vi "From CSV File.vi"(8 "error in (no error)":errorcluster, 9 "Path":path, 10 "engine in":refnum<class "engine configuration.lvclass">, 11 "module editor node in":refnum<class "module editor node.lvclass">) -> (0 "error out":errorcluster, 1 "Update":bool, 2 "engine out":refnum<class "engine configuration.lvclass">, 3 "module editor node out":refnum<class "module editor node.lvclass">)   [LabVIEW 2014, in "PL Framework Configuration Tool.lvlib" / "module editor node.lvclass"]
uses:
  module editor node.lvclass
  <vilib>/NI/Module Execution Interface/Engine Configuration/engine configuration.lvclass
  <vilib>/NI/Tag Bus Module Framework/module configuration/TBM module configuration.lvclass
  <vilib>/NI/Configuration Framework/serializable configuration/NISE_CEF_serializable configuration.lvclass
panel:
  in  "type (empty)":string[][](array[string])
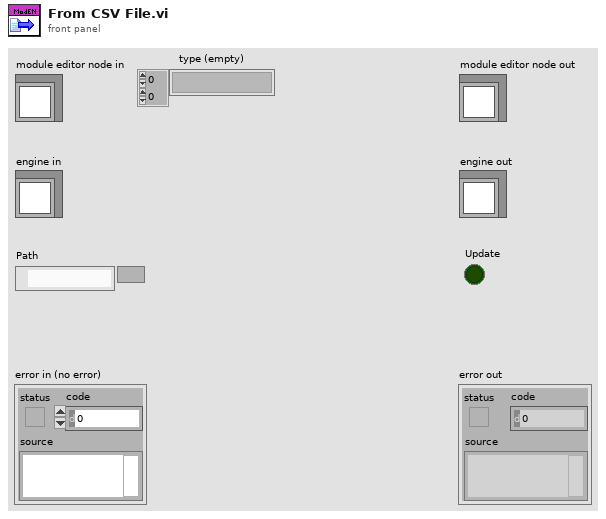
[diagram p1: front panel]
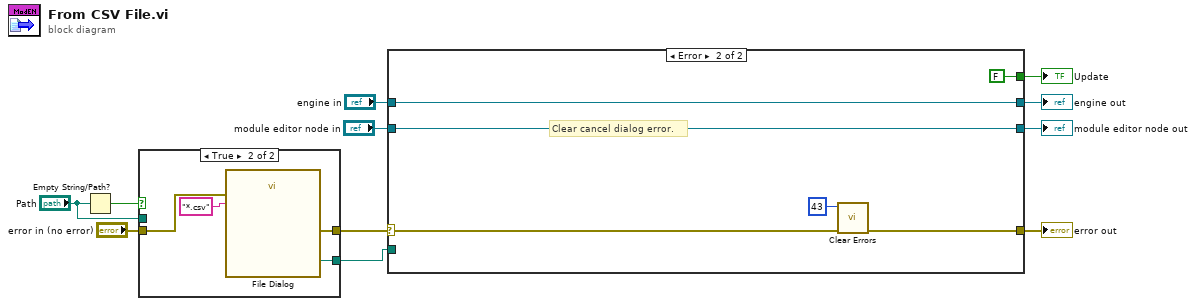
[diagram p0: block diagram]
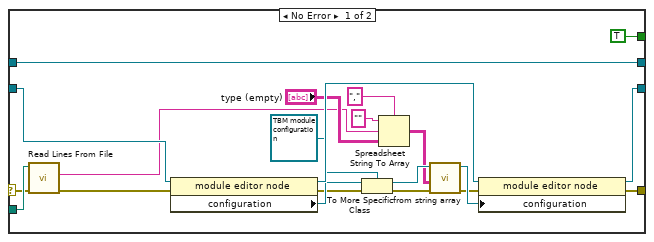
[diagram p3: hidden frame]
diagram:
  n1 = Empty String/Path?(string/path="Path") -> (empty?=w8:bool)
  n2 = case shown="True" w8 {
    tunnel: "error in (no error)" -> [w12 w16]
    tunnel: [w12 w15] -> w6
    tunnel: [w13 w14] -> w5
    tunnel: "Path" -> [w13 _]
    frame False {
    }
    frame True {
      n3 = call "File Dialog"("error in"=w16, "pattern (all files)"="*.csv") -> ("selected path"=w14:path, "error out"=w15:errorcluster)  [unwired: 10 in, 2 out]
    }
  }
  n4 = case shown="Error" w6 {
    selector: w6 -> [w20 w42]
    tunnel: [w27 w41] -> w11
    tunnel: [w36 w44] -> w9
    tunnel: "module editor node in" -> [w38 w44]
    tunnel: w5 -> [w26 _]
    tunnel: "engine in" -> [w18 w39]
    tunnel: [TRUE ("Update") FALSE ("Update")] -> w3
    tunnel: [w18 w39] -> w1
    frame No Error {
      n5 = call "Read Lines From File.vi"("file path (dialog if empty)"=w26, "error in (not an error)"=w20) -> ("line string"=w24:string, "error out"=w19:errorcluster)  [unwired: 5 in, 1 out]
      n6 = property class="module editor node"(reference=w38, error in=w19) -> (reference out=w37:refnum<class "module editor node.lvclass">, error out=w30:errorcluster, "configuration"=w34:refnum<class "NISE_CEF_serializable configuration.lvclass">)
      n7 = To More Specific Class(target class=refnum<class "TBM module configuration.lvclass"> refnum ("module configuration in"), reference=w34, error in=w30) -> (specific class reference=w33:refnum<class "TBM module configuration.lvclass">, error out=w29:errorcluster)
      n8 = Spreadsheet String To Array(delimiter (Tab)=",", format string="", spreadsheet string=w24, array type (2D Dbl)="type (empty)") -> (array=w21:string[][])
      n9 = call-dynamic "from string array.vi"("error in (no error)"=w29, "String Array"=w21, "module configuration in"=w33) -> ("error out"=w28:errorcluster, "module configuration out"=w32:refnum<class "TBM module configuration.lvclass">)  [unwired: 7 in]
      n10 = property class="module editor node"(reference=w37, error in=w28, "configuration"=w32) -> (reference out=w36:refnum<class "module editor node.lvclass">, error out=w27:errorcluster)
    }
    frame Error {
      # "Clear cancel dialog error."
      n11 = call <vilib>:"Clear Errors.vi"("error in (no error)"=w42, "specific error code to clear (0: all)"=43) -> ("error out"=w41:errorcluster)  [unwired: 4 in, 1 out]
    }
  }
  "error out" <- w11
  "module editor node out" <- w9
  "Update" <- w3
  "engine out" <- w1
